vi "version.vi"(7 "LabVIEW Web Service Request":refnum<class "Web Request.lvclass">) -> ()   [LabVIEW 2017]
uses:
  <vilib>/wsapi/Web Request.lvclass
  C:/Program Files (x86)/National Instruments/LabVIEW 2017/vi.lib/wsapi/Web Service.lvclass
  <vilib>/LVH/i3 JSON/JSON Generation/Create Value Files/Create Value - Object.vi
  <vilib>/LVH/i3 JSON/JSON Generation/Add Object Parameter Files/Add Object Parameter - String.vi
  <vilib>/LVH/i3 JSON/i3-json.lvlib
  <vilib>/wsapi/Web Service.lvclass
panel:
  out "error out":errorcluster
  in  "error in (no error)":errorcluster
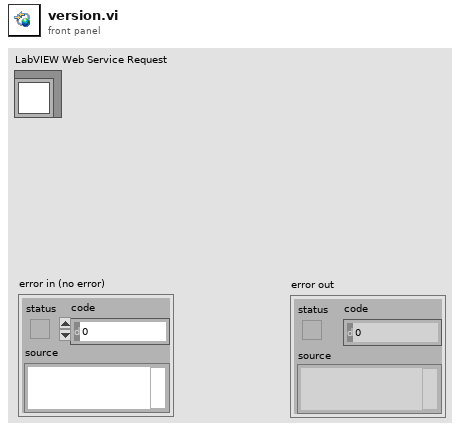
[diagram p1: front panel]
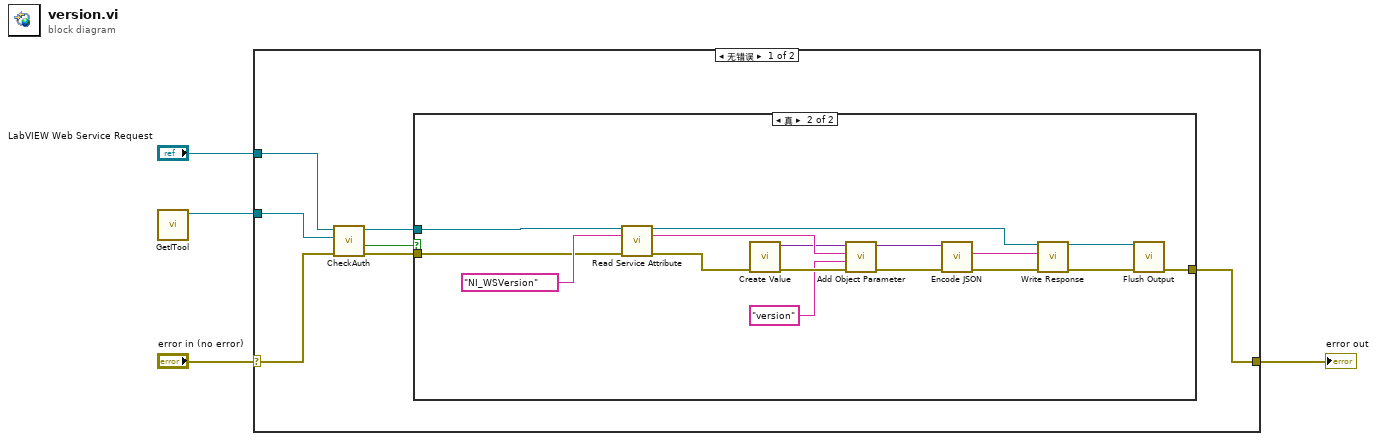
[diagram p0: block diagram]
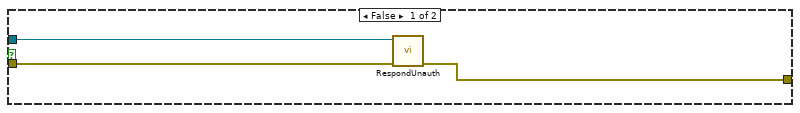
[diagram p2: hidden frame]
diagram:
  n1 = call "GetITool.vi"() -> ("ITool.lvclass out"=w1:refnum<class "ITool.lvclass">)  [unwired: 11 in]
  n2 = case shown="无错误" "error in (no error)" {
    selector: "error in (no error)" -> [w10 w31]
    tunnel: "LabVIEW Web Service Request" -> [w7 _]
    tunnel: [w11 w31] -> w2
    tunnel: w1 -> [w8 _]
    frame No Error {
      n3 = call "CheckAuth.vi"("error in (no error)"=w10, "ITool in"=w8, "LabVIEW Web Service Request"=w7) -> ("error out"=w6:errorcluster, "isAuthrized"=w9:bool, "LabVIEW Web Service Request out"=w5:refnum<class "Web Request.lvclass">)  [unwired: 5 in, 1 out]
      n4 = case shown="真" w9 {
        tunnel: [w12 w30] -> w11
        tunnel: w6 -> [w13 w16]
        tunnel: w5 -> [w14 w15]
        frame False {
          n5 = call "RespondUnauth.vi"("error in (no error)"=w13, "LabVIEW Web Service Request"=w14) -> ("error out"=w12:errorcluster)  [unwired: 9 in]
        }
        frame True {
          n6 = call <vilib>:"Read Service Attribute.vi"("LabVIEW Web Service"=w15, "attribute name"="NI_WSVersion", "error in (no error)"=w16) -> ("LabVIEW Web Service out"=w20:refnum<class "Web Request.lvclass">, "value"=w29:string, "error out"=w21:errorcluster)  [unwired: 10 in]
          n7 = call-poly <vilib>:"Create Value.vi"("error in (no error)"=w21) -> ("error out"=w26:errorcluster, "JSON Tree"=w25:variant)  [unwired: 9 in]
          n8 = call-poly <vilib>:"Add Object Parameter.vi"("error in (no error)"=w26, "Name"="version", "String"=w29, "JSON Tree in (JSON Object)"=w25) -> ("error out"=w27:errorcluster, "JSON Tree out (JSON Object)"=w28:variant)  [unwired: 6 in]
          n9 = call <vilib>:"Encode JSON.vi"("error in (no error)"=w27, "JSON Tree"=w28) -> ("error out"=w22:errorcluster, "String"=w17:string)  [unwired: 4 in]
          n10 = call <vilib>:"Write Response.vi"("LabVIEW Web Service Request"=w20, "response string"=w17, "error in (no error)"=w22) -> ("LabVIEW Web Service Request out"=w18:refnum<class "Web Request.lvclass">, "error out"=w19:errorcluster)  [unwired: 11 in]
          n11 = call <vilib>:"Flush Output.vi"("LabVIEW Web Service Request"=w18, "error in (no error)"=w19) -> ("error out"=w30:errorcluster)  [unwired: 12 in, 1 out]
        }
      }
    }
    frame Error {
    }
  }
  "error out" <- w2
